vi "_Subsystem_Name Controller.vi"(8 "error in":errorcluster) -> ()   [LabVIEW 2023]
doc: "This VI responds to drive commands both auto and tele Opmodes.\nIt owns the drivebase motors and sensors and runs independent from opModes. Commands can run for arbitrary times, but newly posted commands will interupt as long as Check is called and used for time delays."
uses:
  Implementation/_Subsystem_Name Operations.ctl
  Implementation/_Subsystem_Name Setpoints.ctl
  <vilib>/MRC/Types/CmdCtl Completion.ctl
  Implementation/Swerve Support/_Subsystem_Name Global.vi
  <vilib>/REV Custom Controls/Spark Output Control Type.ctl
  <vilib>/REVLibDriver/REVLibDriver.lvlib
  <vilib>/REV Custom Controls/Spark Voltage Compensation.ctl
  <resource>/objmgr/REVSpark.rc
  <vilib>/Rock Robotics/WPI/Framework/Completion Status.ctl
panel:
  in  "Drive Controller Diagnostics":T1(tab)
  out "Swerve Visualizer":cluster{dbl[], dbl[]}[](graph)
  out "Pod Comparisons (Diff -> Setpoint - Actual)":T2
  out "(Calibration) Steering":T3
  in  "Default PID Gains":T4
  in  "Auto Gains":T4={{"P Gain"=0.16, "I Gain"=0.0, "D Gain"=0.0, "kV"=0.78}, "I Zone"=0.0, "Output LImits"={"Min Output"=-1.0, "Max Output"=1.0}}
  in  "Abort Cmd":bool
  in  "Execute Cmd":bool
  in  "Interactive Values":T5
  out "Command Timing":cluster{"Start Time (ms)":u32, "Iterations":i32}
  out "Status":T7
  out "Current Command Data":T5
  out "Cmd Summary":string
  # "Interactive Command: You may fill in the settings for a command\nand schedule it with the Execute button. You can observe and abort\nany command while fine tuning the code for the controller."
  # "The panel for a subsystem is a great place to chart or view operational\nstate of the mechanism. You can also introduce debug-specific operations\nsuch as tuning PID or calibration."
  # "You can place an image of the field here and use picture drawing"
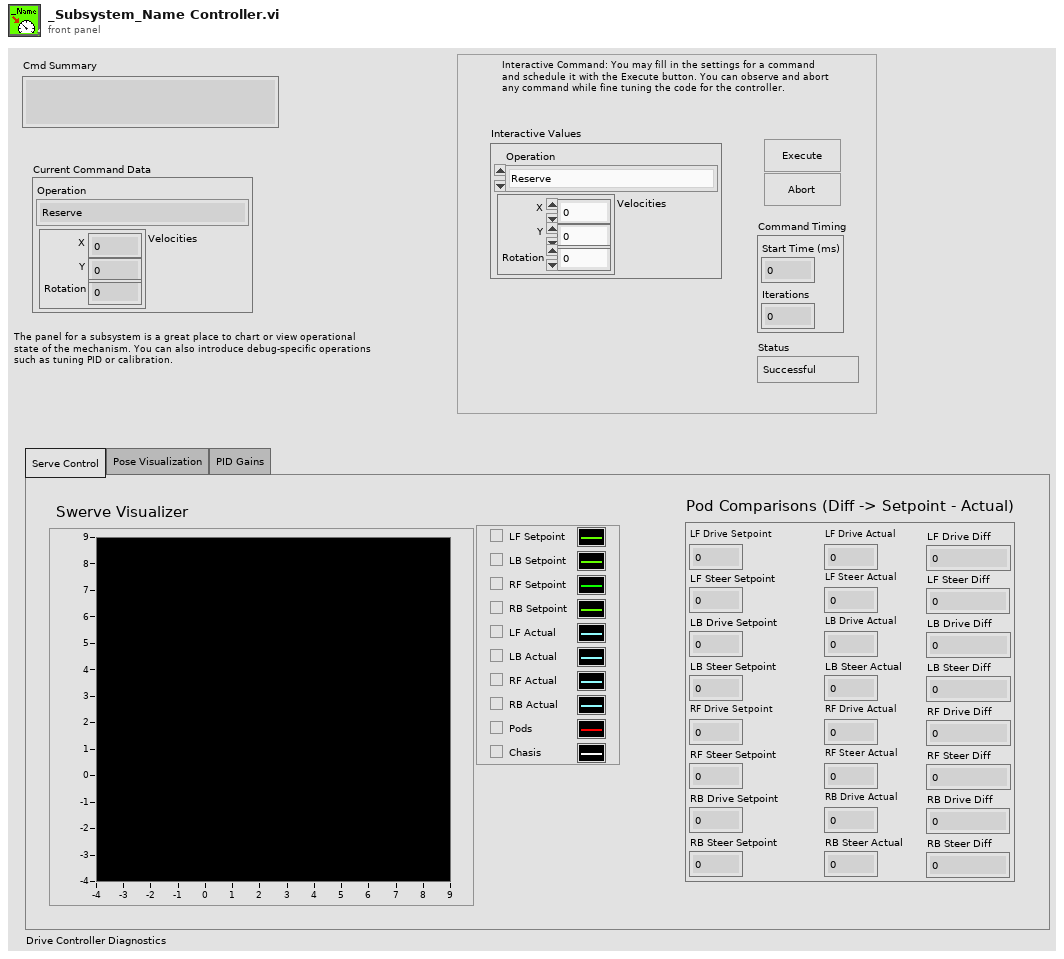
[diagram p1: front panel]
types:
  T1 = enum32{"Serve Control", "Pose Visualization", "PID Gains"}
  T2 = cluster{"LF Drive Setpoint":dbl, "LF Steer Setpoint":dbl, "LB Drive Setpoint":dbl, "LB Steer Setpoint":dbl, "RF Drive Setpoint":dbl, "RF Steer Setpoint":dbl, "RB Drive Setpoint":dbl, "RB Steer Setpoint":dbl, "LF Drive Actual":dbl, "LF Steer Actual":dbl, "LB Drive Actual":dbl, "LB Steer Actual":dbl, "RF Drive Actual":dbl, "RF Steer Actual":dbl, "RB Drive Actual":dbl, "RB Steer Actual":dbl, "LF Drive Diff":dbl, "LF Steer Diff":dbl, "LB Drive Diff":dbl, "LB Steer Diff":dbl, "RF Drive Diff":dbl, "RF Steer Diff":dbl, "RB Drive Diff":dbl, "RB Steer Diff":dbl}
  T3 = cluster{"Left Front":dbl, "Left Back":dbl, "Right Front":dbl, "Right Back":dbl}
  T4 = cluster{cluster{"P Gain":dbl, "I Gain":dbl, "D Gain":dbl, "kV":dbl}, "I Zone":dbl, "Output LImits":cluster{"Min Output":dbl, "Max Output":dbl}}
  T5 = typedef "_Subsystem_Name Setpoints.ctl" = cluster{"Operation":T6, "Velocities":cluster{"X":dbl, "Y":dbl, "Rotation":dbl}}
  T6 = typedef "_Subsystem_Name Operations.ctl" = enum16{"Reserve", "Read Current", "Immediate", "Auto", "Calibrate", "Config for Auto", "Config for TeleOp"}
  T7 = typedef "Completion Status.ctl" = enum16{"Successful", "Aborted", "Incomplete"}
  T8 = typedef "(NEO-NEO-ThroughBore-Pigeon2) Swerve.ctl" = cluster{"Drive Motor IDs":cluster{"[0]":T9, "[1]":T9, "[2]":T9, "[3]":T9}, "Steer Motor IDs":cluster{"[0]":T9, "[1]":T9, "[2]":T9, "[3]":T9}, "Pod Locations (ft)":T10, "Drive Scaling":dbl, "Steer Scaling":dbl}
  T9 = typedef "REVLibDriver.lvlib/REVSparkRefnum.ctl" = refnum<k20>
  T10 = typedef "Pod Positions.ctl" = cluster{"Left Front":dbl[], "Left Back":dbl[], "Right Front":dbl[], "Right Back":dbl[]}
  T11 = typedef "Command Status Info.ctl" = cluster{"Name":string, "Status":T7, "notifier out":T12}
  T12 = typedef "Completion Notifier.ctl" = refnum<notifier>
  T13 = cluster{"Current Command":T5, "Command Timing":cluster{"Start Time (ms)":u32, "Iterations":i32}, "Command Arguments":cluster{"Command Info":T11, "Description":string, "Default Command":T5, "queue out":refnum<queue>, "Subsystem Name":string}}
  T14 = typedef "CmdCtl Completion.ctl" = enum16{"incomplete", "finished"}
  T15 = typedef "REVLibDriver.lvlib/Spark Voltage Compensation.ctl" = cluster{"Mode":u32, "Nominal Voltage":dbl}
  T16 = typedef "Drive Conditions.ctl" = cluster{"Field Centric":bool, "Reset PIDs":bool}
  T17 = typedef "REVLibDriver.lvlib/Spark Output Control Type.ctl" = enum16{"Percent VBus", "Velocity", "Voltage", "Position", "Current", "MAXMotion Position", "MAXMotion Velocity"}
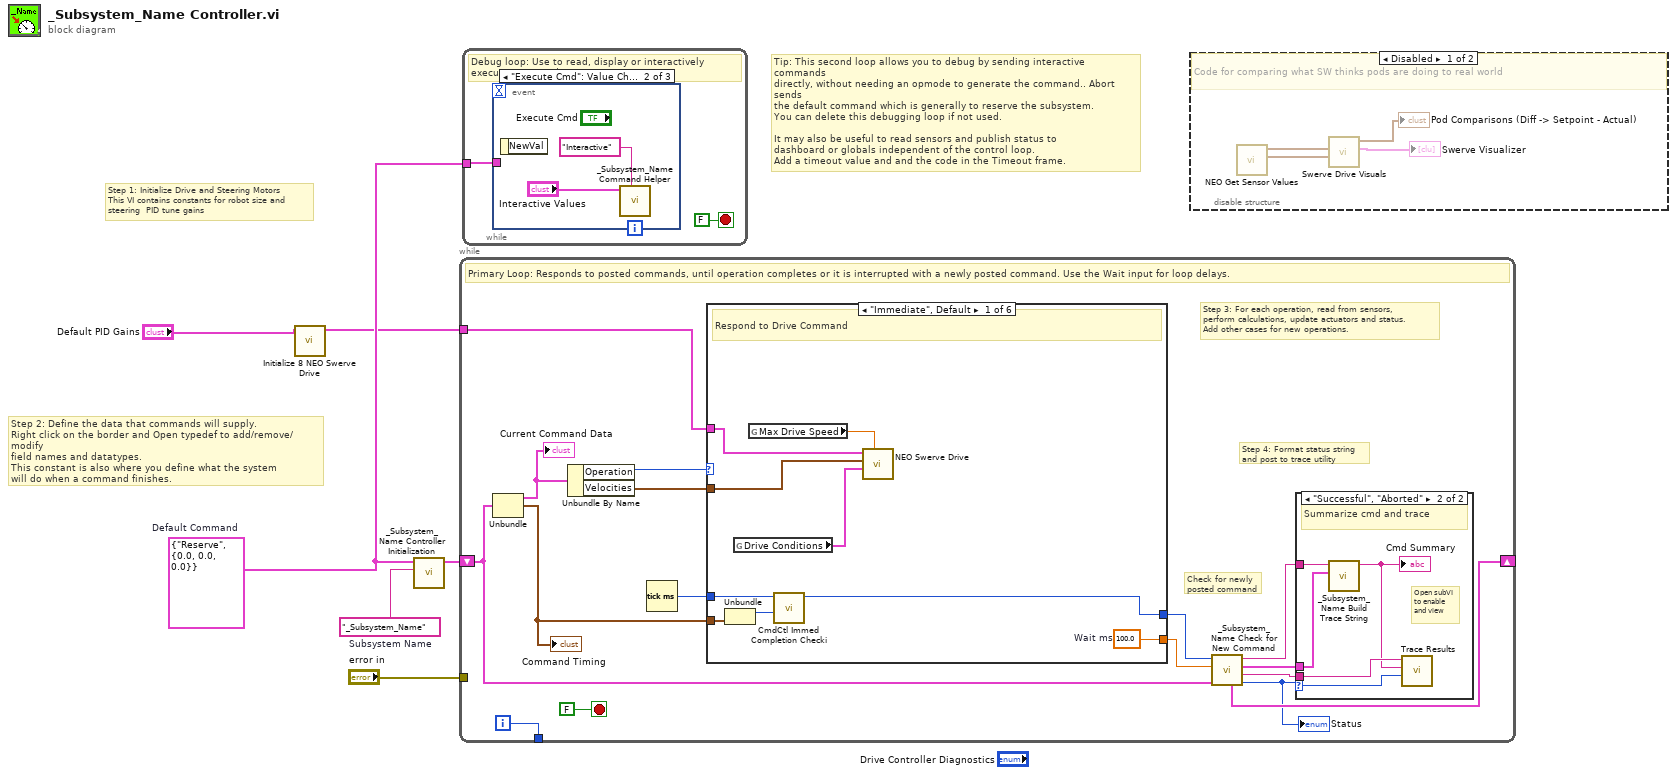
[diagram p0: block diagram]
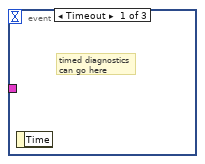
[diagram p3: hidden frame]
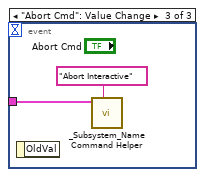
[diagram p4: hidden frame]
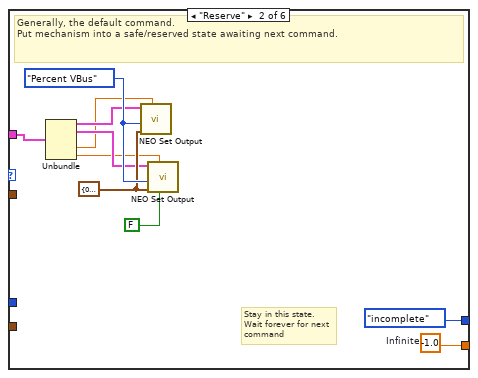
[diagram p6: hidden frame]
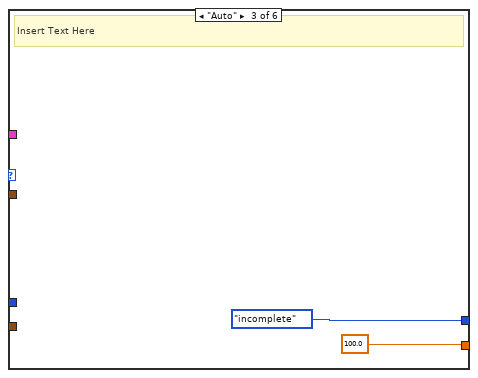
[diagram p7: hidden frame]
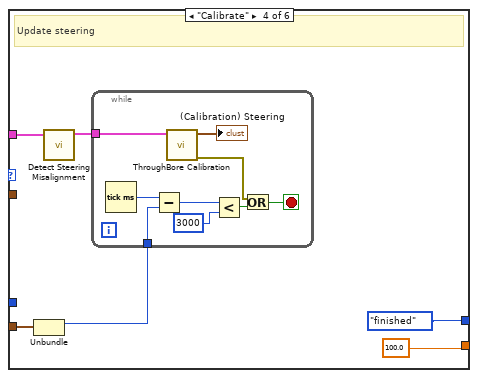
[diagram p8: hidden frame]
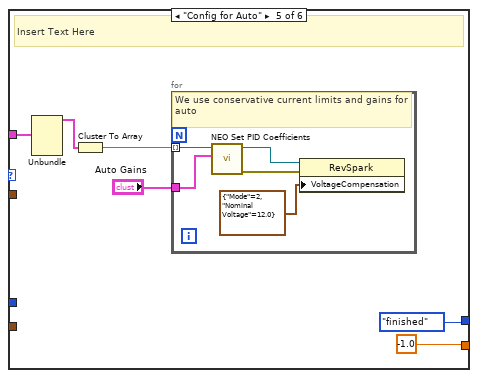
[diagram p9: hidden frame]
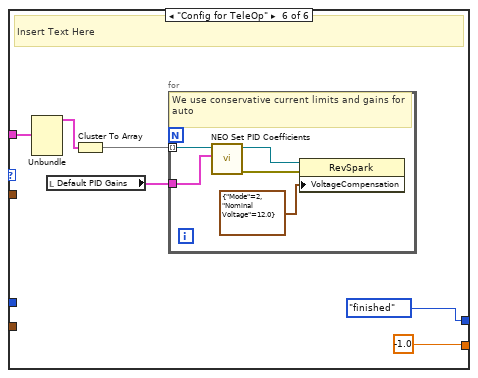
[diagram p10: hidden frame]
diagram:
  w3 = T5 {"Operation"=enum."Reserve", "Velocities"={"X"=0.0, "Y"=0.0, "Rotation"=0.0}}  # Default Command
  w4 = "_Subsystem_Name"  # Subsystem Name
  # "Tip: This second loop allows you to debug by sending interactive commands\ndirectly, without needing an opmode to generate the command.. Abort sends\nthe default command which is generally to reserve the subsystem.\nYou can delete this debugging loop if not used.\n\nIt may also be useful to read sensors and publish status to\ndashboard or globals independent of the control loop.\nAdd a timeout value and and the code in the Timeout frame."
  # "Step 2: Define the data that commands will supply.\nRight click on the border and Open typedef to add/remove/modify\nfield names and datatypes.\nThis constant is also where you define what the system\nwill do when a command finishes."
  # "Step 1: Initialize Drive and Steering Motors\nThis VI contains constants for robot size and\nsteering  PID tune gains"
  n1 = call "Initialize 8 NEO Swerve Drive.vi"("Drive PID Gains"="Default PID Gains") -> ("(N-N-C-P) Swerve Motors"=w2:T8)  [unwired: 9 in, 1 out]
  n2 = call "_Subsystem_Name Controller Initialization.vi"("Subsystem Name"=w4, "Default Command"=w3) -> ("Current Command"=w5:T13)  [unwired: 9 in]
  n3 = while {
    shift-right: [w17] -> _
    shift-left: w5 -> [w11]
    tunnel: [w21] -> _
    tunnel: "error in" -> [_]
    tunnel: w2 -> [w7]
    i -> [w21]
    stop <- FALSE stop-if-true
    # "Step 4: Format status string\nand post to trace utility"
    # "Check for newly\nposted command"
    # "Step 3: For each operation, read from sensors,\nperform calculations, update actuators and status.\nAdd other cases for new operations."
    # "Primary Loop: Responds to posted commands, until operation completes or it is interrupted with a newly posted command. Use the Wait input for loop delays."
    n4 = Unbundle(w11) -> ("Current Command"=w9:T5, "Command Timing"=w10:cluster{"Start Time (ms)":u32, "Iterations":i32})  [unwired: 1 out]
    "Command Timing" <- w10
    "Current Command Data" <- w9
    n5 = Unbundle By Name(w9) -> ("Operation"=w20:T6, "Velocities"=w19:cluster{"X":dbl, "Y":dbl, "Rotation":dbl})
    n6 = Tick Count (ms)() -> (millisecond timer value=w18:u32)
    n7 = case shown="\"Immediate\", Default" w20 {
      tunnel: [w36 w46 100.0 ("Infinite") 100.0 ("Infinite") -1.0 ("Infinite") -1.0 ("Infinite")] -> w15
      tunnel: [w33 CmdCtl_Completion."incomplete" CmdCtl_Completion."incomplete" CmdCtl_Completion."finished" CmdCtl_Completion."finished" CmdCtl_Completion."finished"] -> w16
      tunnel: w10 -> [w35 _ _ w52 _ _]
      tunnel: w19 -> [w28 _ _ _ _ _]
      tunnel: w18 -> [w34 _ _ _ _ _]
      tunnel: w7 -> [w31 w41 _ w50 w68 w79]
      frame "Immediate", Default {
        w36 = 100.0  # Wait ms
        # "Respond to Drive Command"
        n8 = Unbundle(w35) -> ("Start Time (ms)"=w32:u32)  [unwired: 1 out]
        n9 = global read "_Subsystem_Name Global.vi" "Drive Conditions"() -> (w30:T16)
        n10 = global read "_Subsystem_Name Global.vi" "Max Drive Speed"() -> (w29:dbl)
        n11 = call <vilib>:"CmdCtl Immed Completion Checki.vi"("Start Time (ms)"=w32, "current time (ms)"=w34) -> ("Completion"=w33:T14)  [unwired: 9 in]
        n12 = call "NEO Swerve Drive.vi"("Max V"=w29, "Drive Conditions"=w30, "Robot Velocities"=w28, "Motors In"=w31) -> ()  [unwired: 6 in, 2 out]
      }
      frame "Reserve" {
        w43 = T3 {"Left Front"=0.0, "Left Back"=0.0, "Right Front"=0.0, "Right Back"=0.0} ("Arbitrary Feedforward")
        w44 = Spark_Output_Control_Type."Percent VBus" ("Control Mode")
        w46 = -1.0  # Infinite
        # "Stay in this state.\nWait forever for next\ncommand"
        # "Generally, the default command.\nPut mechanism into a safe/reserved state awaiting next command."
        n13 = Unbundle(w41) -> ("Drive Motor IDs"=w40:cluster{"[0]":T9, "[1]":T9, "[2]":T9, "[3]":T9}, "Steer Motor IDs"=w39:cluster{"[0]":T9, "[1]":T9, "[2]":T9, "[3]":T9}, "Drive Scaling"=w37:dbl, "Steer Scaling"=w38:dbl)  [unwired: 1 out]
        n14 = call "NEO Set Output.vi"("Scaling"=w37, "Arbitrary Feedforward"=w43, "Control Mode"=w44, "Motors"=w40) -> ()  [unwired: 7 in, 1 out]
        n15 = call "NEO Set Output.vi"("Add Angle Offsets?"=FALSE, "Scaling"=w38, "Arbitrary Feedforward"=w43, "Control Mode"=w44, "Motors"=w39) -> ()  [unwired: 6 in, 1 out]
      }
      frame "Auto" {
        # "Insert Text Here"
      }
      frame "Calibrate" {
        # "Update steering"
        n16 = Unbundle(w52) -> ("Start Time (ms)"=w51:u32)  [unwired: 1 out]
        n17 = call "Detect Steering Misalignment.vi"("Motors In"=w50) -> ("Motors out"=w49:T8)  [unwired: 10 in]
        n18 = while {
          tunnel: w51 -> [w62]
          tunnel: w49 -> [w58]
          stop <- w55 stop-if-true
          n19 = Tick Count (ms)() -> (millisecond timer value=w63:u32)
          n20 = Subtract(x=w63, y=w62) -> (x-y=w60:u32)
          n21 = call "ThroughBore Calibration.vi"("(N-N-C-P) Swerve Motors"=w58) -> ("error out"=w56:errorcluster, "Steering Angles"=→"(Calibration) Steering":cluster{"LF":dbl, "LB":dbl, "RF":dbl, "RB":dbl})  [unwired: 9 in]
          n22 = Less?(x=w60, y=u32 3000) -> (x < y?=w57:bool)
          n23 = Or(x=w56, y=w57) -> (x .or. y?=w55:bool)
        }
      }
      frame "Config for Auto" {
        # "Insert Text Here"
        n24 = Unbundle(w68) -> ("Drive Motor IDs"=w69:cluster{"[0]":T9, "[1]":T9, "[2]":T9, "[3]":T9})  [unwired: 4 out]
        n25 = Cluster To Array(cluster=w69) -> (array=w67:T9[])
        n26 = for {
          tunnel: w67 -> [w74] mode=indexing
          tunnel: "Auto Gains" -> [w70]
          # "We use conservative current limits and gains for auto"
          n27 = call "NEO Set PID Coefficients.vi"("PID Gains"=w70, "Spark refnum"=w74) -> ("error out"=w71:errorcluster, "Spark refnum out"=w73:T9)  [unwired: 6 in]
          n28 = property class="RevSpark"(reference=w73, error in=w71, "VoltageCompensation"=T15 {"Mode"=2, "Nominal Voltage"=12.0}) -> ()  [unwired: 2 out]
        }
      }
      frame "Config for TeleOp" {
        # "Insert Text Here"
        n29 = Unbundle(w79) -> ("Drive Motor IDs"=w80:cluster{"[0]":T9, "[1]":T9, "[2]":T9, "[3]":T9})  [unwired: 4 out]
        n30 = local read "Default PID Gains"() -> (w77:T4)
        n31 = Cluster To Array(cluster=w80) -> (array=w78:T9[])
        n32 = for {
          tunnel: w78 -> [w85] mode=indexing
          tunnel: w77 -> [w81]
          # "We use conservative current limits and gains for auto"
          n33 = call "NEO Set PID Coefficients.vi"("PID Gains"=w81, "Spark refnum"=w85) -> ("error out"=w82:errorcluster, "Spark refnum out"=w84:T9)  [unwired: 6 in]
          n34 = property class="RevSpark"(reference=w84, error in=w82, "VoltageCompensation"=T15 {"Mode"=2, "Nominal Voltage"=12.0}) -> ()  [unwired: 2 out]
        }
      }
    }
    n35 = call "_Subsystem_Name Check for New Command.vi"("Current Command"=w11, "Wait time (ms)"=w15, "Completion"=w16) -> ("Completion"=w8:T7, "Subsystem Name"=w12:string, "Current Command"=w13:T5, "Initial Trace String"=w14:string, "NextCommand"=w17:T13)  [unwired: 4 in]
    "Status" <- w8
    n36 = case shown="\"Successful\", \"Aborted\"" w8 {
      selector: w8 -> [_ w27]
      tunnel: w14 -> [_ w25]
      tunnel: w13 -> [_ w24]
      tunnel: w12 -> [_ w26]
      frame "Incomplete", Default {
        # "Continuing current command"
      }
      frame "Successful", "Aborted" {
        # "Open subVI\nto enable\nand view"
        # "Summarize cmd and trace"
        n37 = call "_Subsystem_Name Build Trace String.vi"("Current Command"=w24, "Initial Trace String"=w25) -> ("Trace String"=w23:string)  [unwired: 9 in]
        "Cmd Summary" <- w23
        n38 = call <vilib>:"Trace Results.vi"("Status of previous command"=w27, "Description"=w23, "Subsystem"=w26) -> ()  [unwired: 9 in]
      }
    }
  }
  n39 = while {
    tunnel: w3 -> [w86]
    stop <- FALSE stop-if-true
    # "Debug loop: Use to read, display or interactively execute commands."
    n40 = event shown="[1] \"Execute Cmd\": Value Change" {
      selector: _ -> [_ _ _]
      dyn-events: _ -> [_ _ _]
      timeout: _ -> [_ _ _]
      tunnel: w86 -> [_ _ w91]
      event Timeout {
        # "timed diagnostics\ncan go here"
        # "Insert Text Here"
        n41 = event-data() -> ()  [unwired: 1 in, 1 out]
      }
      event "Execute Cmd": Value Change {
        # "Execute"
        n42 = event-data() -> ()  [unwired: 1 in, 1 out]
        n43 = call "_Subsystem_Name Command Helper.vi"("Description"="Interactive", "SubSystem Data"="Interactive Values") -> ()  [unwired: 7 in, 3 out]
      }
      event "Abort Cmd": Value Change {
        # "Insert Text Here"
        n44 = event-data() -> ()  [unwired: 1 in, 1 out]
        n45 = call "_Subsystem_Name Command Helper.vi"("Description"="Abort Interactive", "SubSystem Data"=w91) -> ()  [unwired: 7 in, 3 out]
      }
    }
  }
  n46 = disable-structure shown="Disabled" {
    frame Disabled {
      # "Code for comparing what SW thinks pods are doing to real world"
      n47 = call "NEO Get Sensor Values.vi"() -> ("Steer Angles (degrees)"=w94:T3, "Drive Velocities (ft/s)"=w95:T3)  [unwired: 10 in]
      n48 = call "Swerve Drive Visuals.vi"("Steer Angles (degrees)"=w94, "Drive Velocities (ft/s)"=w95) -> ("Swerve Visualizer"=→"Swerve Visualizer":cluster{dbl[], dbl[]}[], "Pod Comparisons (Diff -> Setpoint - Actual)"=→"Pod Comparisons (Diff -> Setpoint - Actual)":T2)  [unwired: 8 in]
    }
    frame Enabled {
      # "Insert Text Here"
    }
  }
